vi "Set Logger Enqueuer.vi"(8 "error in":errorcluster, 10 "Logger":refnum<class "Message Enqueuer.lvclass">, 11 "LV File Creator in":refnum<class "LV File Creator.lvclass">) -> (0 "error out":errorcluster, 3 "LV File Creator out":refnum<class "LV File Creator.lvclass">)   [LabVIEW 2026, in "LV File Creator.lvclass"]
doc: "Set the logger enqueuer for a Logger Client."
uses:
  LV File Creator.lvclass
  <vilib>/ActorFramework/Message Enqueuer/Message Enqueuer.lvclass
  LV File Creator.lvclass/LV File Creator.ctl
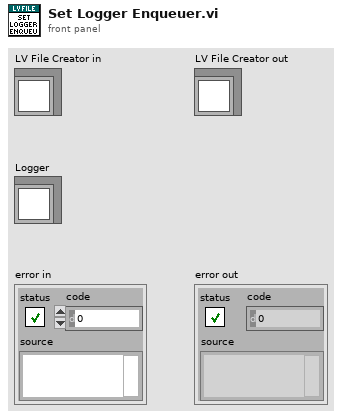
[diagram p1: front panel]
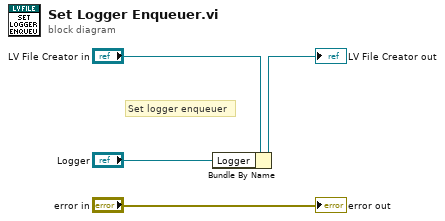
[diagram p0: block diagram]
diagram:
  # "Set logger enqueuer"
  n1 = Bundle By Name(cluster="LV File Creator in", "Logger"="Logger") -> (→"LV File Creator out":refnum<class "LV File Creator.lvclass">)
  "error out" <- "error in"
